vi "update Remote Display.vi"(8 "error in (no error)":errorcluster, 10 "Remote Display On?":bool, 11 "FSV-40N in":refnum<class "FSV-40N.lvclass">) -> (0 "error out":errorcluster, 3 "FSV-40N out":refnum<class "FSV-40N.lvclass">)   [LabVIEW 2023, in "Spectrum Analyzer.lvlib" / "FSV-40N.lvclass"]
uses:
  FSV-40N.lvclass
  FSV-40N.lvclass/FSV-40N.ctl
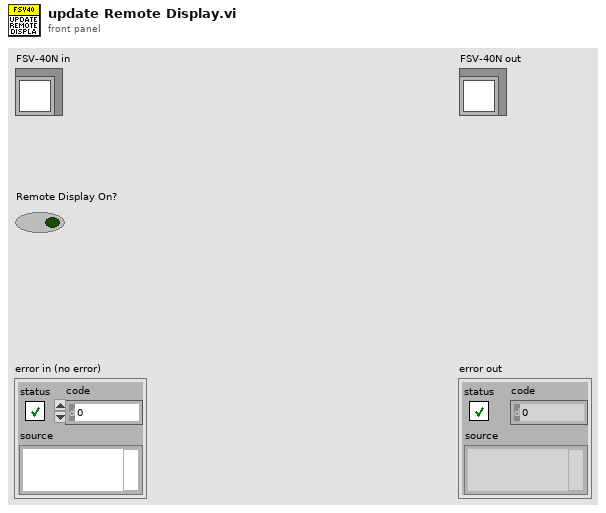
[diagram p1: front panel]
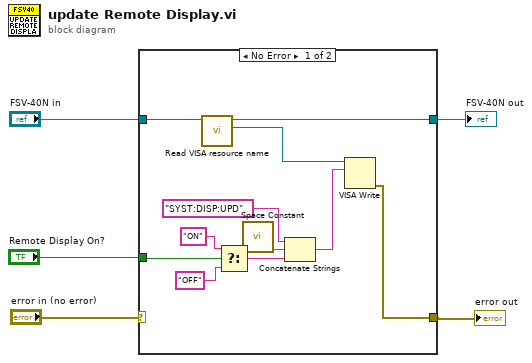
[diagram p0: block diagram]
diagram:
  n1 = case shown="No Error" "error in (no error)" {
    selector: "error in (no error)" -> [_ w17]
    tunnel: "FSV-40N in" -> [w16 w18]
    tunnel: [w6 w18] -> w3
    tunnel: [w7 w17] -> w2
    tunnel: "Remote Display On?" -> [w14 _]
    frame No Error {
      n2 = call "Read VISA resource name.vi"("FSV-40N in"=w16) -> ("VISA resource name"=w15:refnum<visa-resource-name>, "FSV-40N out"=w6:refnum<class "FSV-40N.lvclass">)  [unwired: 8 in, 1 out]
      n3 = Select(t="ON", s=w14, f="OFF") -> (s? t:f=w11:string)
      n4 = call <vilib>:"Space Constant.vi"() -> ("String"=w9:string)
      n5 = Concatenate Strings("SYST:DISP:UPD" ("string"), w9, w11) -> (w8:string)
      n6 = VISA Write(VISA resource name=w15, write buffer=w8) -> (error out=w7:errorcluster)  [unwired: 1 in, 2 out]
    }
    frame Error {
    }
  }
  "error out" <- w2
  "FSV-40N out" <- w3
